vi "Read Waiting Time(ms).vi"(8 "error in (no error)":errorcluster, 11 "NR in":refnum<class "NR.lvclass">) -> (0 "error out":errorcluster, 2 "Waiting Time(ms)":u32, 3 "NR out":refnum<class "NR.lvclass">)   [LabVIEW 2023, in "ANRITSU Call Box.lvlib" / "NR.lvclass"]
uses:
  NR.lvclass
  NR.lvclass/NR.ctl
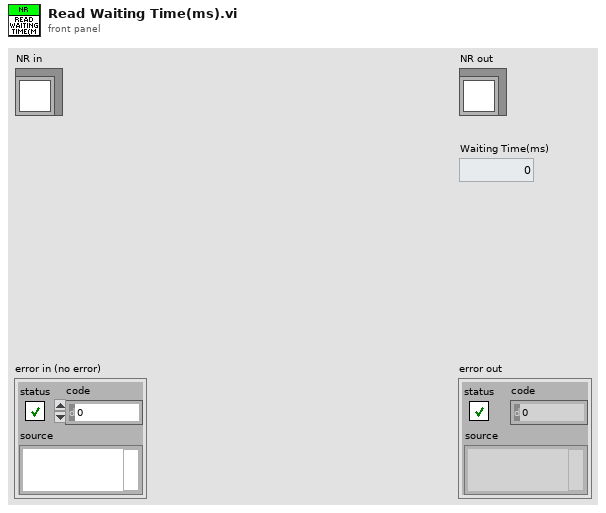
[diagram p1: front panel]
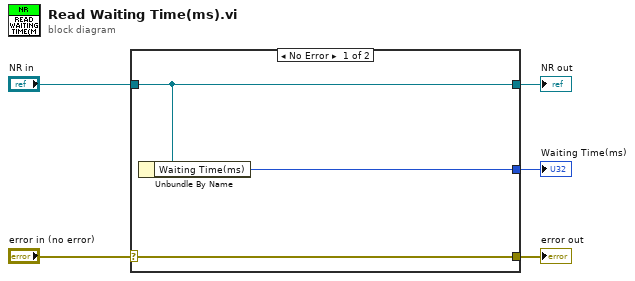
[diagram p0: block diagram]
diagram:
  n1 = case shown="No Error" "error in (no error)" {
    selector: "error in (no error)" -> [w8 w9]
    tunnel: [w8 w9] -> w4
    tunnel: [w7 w10] -> w2
    tunnel: "NR in" -> [w7 w10]
    tunnel: [w6 _] -> w1
    frame No Error {
      n2 = Unbundle By Name(w7) -> ("Waiting Time(ms)"=w6:u32)
    }
    frame Error {
    }
  }
  "error out" <- w4
  "NR out" <- w2
  "Waiting Time(ms)" <- w1
